vi "Add Result Fields.vi"(8 "error in":errorcluster, 9 "serverInfo":string, 10 "method":string, 11 "response":string) -> (0 "error out":errorcluster, 3 "response out":string)   [LabVIEW 2020, in "MCP Server.lvlib"]
doc: "Adds the result fields of MCP 2026-07-28 to a JSON-RPC response that has a result: \"resultType\":\"complete\", and serverInfo under _meta \"io.modelcontextprotocol/serverInfo\" (into an existing _meta, or as a new _meta). For the methods named in Cache Hints.vi it also sets ttlMs and cacheScope (Add Cache Hints.vi). Used by Complete Handler Result.vi.\n\nRuns regardless of error in, which is passed through unchanged; the JSONtext errors are not passed on."
uses:
  MCP Server.lvlib
  <vilib>/JDP Science/JSONtext/Next JSON Value.vi
  <vilib>/JDP Science/JSONtext/String Subset.vi
  <vilib>/JDP Science/JSONtext/Parsing/Advance past next JSON Value (inlined COPY).vi
  <vilib>/JDP Science/JSONtext/Parsing/Advance past whitespace.vi
  <vilib>/JDP Science/JSONtext/Parsing/Advance past String.vi
  <vilib>/JDP Science/JSONtext/Parsing/Advance past Number.vi
  <vilib>/JDP Science/JSONtext/Parsing/Advance past Line Ending.vi
  <vilib>/JDP Science/JSONtext/Parsing/Parse Full Path or Item Name.vi
  <vilib>/JDP Science/JSONtext/Parsing/Advance past Array.vi
  <vilib>/JDP Science/JSONtext/Parsing/Advance past Object.vi
  <vilib>/JDP Science/JSONtext/support/Error Cluster From Code.vi
  <vilib>/JDP Science/JSONtext/Offset/Find Item Locations by Path.vi
  <vilib>/JDP Science/JSONtext/JSONtext.lvlib
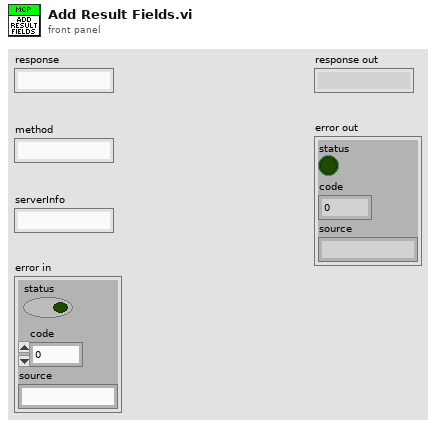
[diagram p1: front panel]
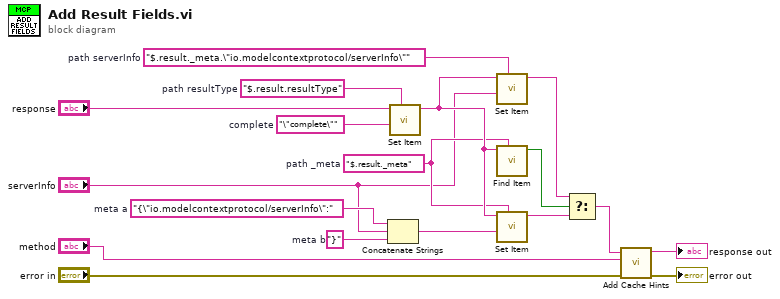
[diagram p0: block diagram]
diagram:
  w10 = "}"  # meta b
  w9 = "{\"io.modelcontextprotocol/serverInfo\":"  # meta a
  w8 = "$.result._meta.\"io.modelcontextprotocol/serverInfo\""  # path serverInfo
  w7 = "$.result._meta"  # path _meta
  w6 = "\"complete\""  # complete
  w5 = "$.result.resultType"  # path resultType
  n1 = Concatenate Strings(w9, "serverInfo", w10) -> (w13:string)
  n2 = call <vilib>:"Set Item.vi"("$Path or Item Name"=w5, "JSON to Insert"=w6, "JSON"="response") -> ("<JSON>"=w11:string)  [unwired: 5 in, 2 out]
  n3 = call <vilib>:"Set Item.vi"("$Path or Item Name"=w8, "JSON to Insert"="serverInfo", "JSON"=w11) -> ("<JSON>"=w14:string)  [unwired: 5 in, 2 out]
  n4 = call <vilib>:"Find Item.vi"("$Path or Item Name"=w7, "JSON"=w11) -> ("Found"=w12:bool)  [unwired: 6 in, 3 out]
  n5 = call <vilib>:"Set Item.vi"("$Path or Item Name"=w7, "JSON to Insert"=w13, "JSON"=w11) -> ("<JSON>"=w15:string)  [unwired: 5 in, 2 out]
  n6 = Select(t=w14, s=w12, f=w15) -> (s? t:f=w16:string)
  n7 = call "Add Cache Hints.vi"("error in"="error in", "method"="method", "response"=w16) -> ("error out"=→"error out":errorcluster, "response out"=→"response out":string)  [unwired: 7 in]
